vi "Tool Object.vi"(8 "error in (no error)":errorcluster, 11 "Tool Rectangle in":refnum<class "Tool Rectangle.lvclass">) -> (0 "error out":errorcluster, 3 "Tool Rectangle out":refnum<class "Tool Rectangle.lvclass">)   [LabVIEW 2019, in "Tool Rectangle.lvclass"]
uses:
  Tool Rectangle.lvclass
  Settings/ObjectSettings/ObjectSettings.lvclass/ObjectSettings.ctl
  Settings/Rectangle Settings/Rectangle Settings.lvclass
  C:/Users/Albro/Documents/GitHub/AFM-Lithography/lvsrc/Classes/Settings/ObjectSettings/ObjectSettings.lvclass
  Parse/Rectangle/Rectangle.lvclass
  Settings/ObjectSettings/ObjectSettings.lvclass
panel:
  out "XY Graph":cluster{"X":dbl, "Y":dbl}[](graph)
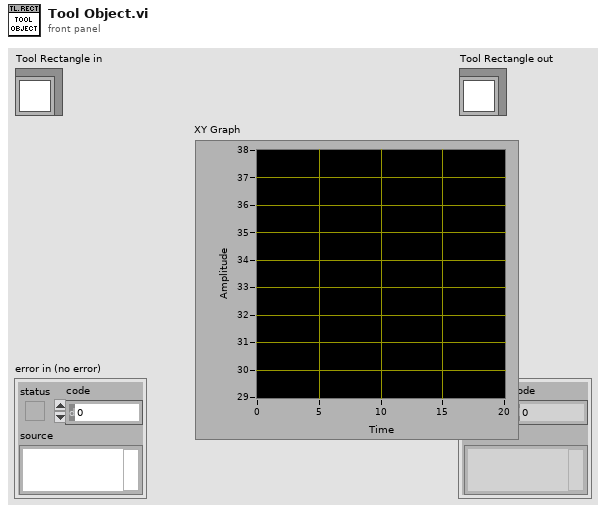
[diagram p1: front panel]
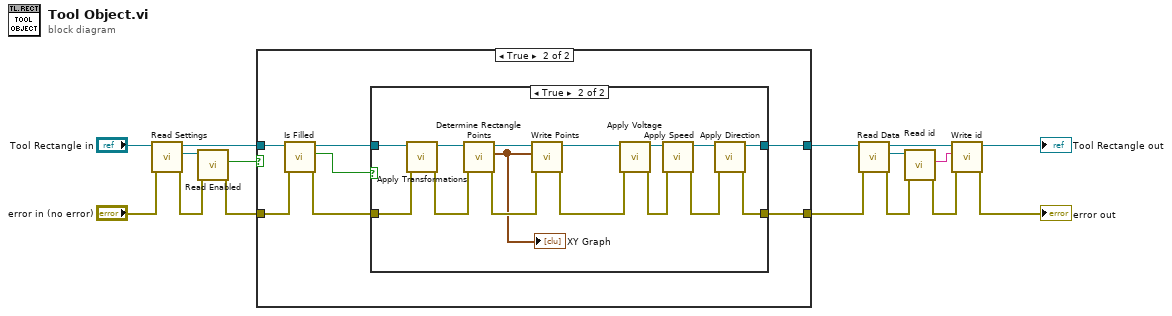
[diagram p0: block diagram]
diagram:
  n1 = call-dynamic "Read Settings.vi"("error in (no error)"="error in (no error)", "Tool Rectangle in"="Tool Rectangle in") -> ("error out"=w11:errorcluster, "Rectangle Settings.lvclass"=w12:refnum<class "Rectangle Settings.lvclass">, "Tool Rectangle out"=w13:refnum<class "Tool Rectangle.lvclass">)  [unwired: 7 in]
  n2 = call "Read Enabled.vi"("error in (no error)"=w11, "ObjectSettings in"=w12) -> ("error out"=w15:errorcluster, "Enabled"=w16:bool)  [unwired: 7 in, 1 out]
  n3 = case shown="True" w16 {
    tunnel: w13 -> [w18 w25]
    tunnel: [w18 w20] -> w4
    tunnel: w15 -> [w17 w23]
    tunnel: [w17 w19] -> w2
    frame False {
    }
    frame True {
      n4 = call-dynamic "Is Filled.vi"("error in (no error)"=w23, "Tool Rectangle in"=w25) -> ("error out"=w22:errorcluster, "x != y?"=w21:bool, "Tool Rectangle out"=w24:refnum<class "Tool Rectangle.lvclass">)  [unwired: 7 in]
      n5 = case shown="True" w21 {
        tunnel: w24 -> [w27 w42]
        tunnel: [w27 w34] -> w20
        tunnel: [w26 w29] -> w19
        tunnel: w22 -> [w26 w41]
        frame False {
          # "#TODO\nAdd unfilled rectangles"
        }
        frame True {
          n6 = call-dynamic "Apply Transformations.vi"("error in (no error)"=w41, "Tool Rectangle in"=w42) -> ("error out"=w39:errorcluster, "Tool Rectangle out"=w40:refnum<class "Tool Rectangle.lvclass">)  [unwired: 8 in]
          n7 = call-dynamic "Determine Rectangle Points.vi"("error in (no error)"=w39, "Tool Rectangle in"=w40) -> ("error out"=w37:errorcluster, "interleaved array"=w28:cluster{"X":dbl, "Y":dbl}[], "Tool Rectangle out"=w38:refnum<class "Tool Rectangle.lvclass">)  [unwired: 7 in]
          "XY Graph" <- w28
          n8 = call-dynamic "Write Points.vi"("error in (no error)"=w37, "Points"=w28, "Tool Object in"=w38) -> ("error out"=w32:errorcluster, "Tool Object out"=w36:refnum<class "Tool Rectangle.lvclass">)  [unwired: 7 in]
          n9 = call-dynamic "Apply Voltage.vi"("error in (no error)"=w32, "Tool Rectangle in"=w36) -> ("error out"=w31:errorcluster, "Tool Rectangle out"=w35:refnum<class "Tool Rectangle.lvclass">)  [unwired: 8 in]
          n10 = call-dynamic "Apply Speed.vi"("error in (no error)"=w31, "Tool Rectangle in"=w35) -> ("error out"=w30:errorcluster, "Tool Rectangle out"=w33:refnum<class "Tool Rectangle.lvclass">)  [unwired: 8 in]
          n11 = call-dynamic "Apply Direction.vi"("error in (no error)"=w30, "Tool Rectangle in"=w33) -> ("error out"=w29:errorcluster, "Tool Rectangle out"=w34:refnum<class "Tool Rectangle.lvclass">)  [unwired: 8 in]
        }
      }
    }
  }
  n12 = call-dynamic "Read Data.vi"("error in (no error)"=w2, "Tool Rectangle in"=w4) -> ("error out"=w6:errorcluster, "Rectangle.lvclass"=w9:refnum<class "Rectangle.lvclass">, "Tool Rectangle out"=w8:refnum<class "Tool Rectangle.lvclass">)  [unwired: 7 in]
  n13 = call-dynamic "Read id.vi"("error in (no error)"=w6, "Rectangle in"=w9) -> ("error out"=w5:errorcluster, "id"=w7:string)  [unwired: 7 in, 1 out]
  n14 = call-dynamic "Write id.vi"("error in (no error)"=w5, "id"=w7, "Tool Object in"=w8) -> ("error out"=→"error out":errorcluster, "Tool Object out"=→"Tool Rectangle out":refnum<class "Tool Rectangle.lvclass">)  [unwired: 7 in]
